vi "主VI.vi"() -> ()   [LabVIEW 2011]
panel:
  in  "长度":dbl=250.0
  out "Data":dbl[](array[numeric])
  out "Out":string=" "
  in  "退出":bool
  out "会话":u32
  in  "超时":u32=2000
  in  "地址":string="[C:DSO][D:DSO-2202M][T:USB][PID:0x834][VID:0x5656][EI:0x82][EO:0x4][CFG:1][I:0] DSO-2202M DSO-2202M"
  in  "读指令":string="dconfig;"
  in  "写指令":string="key:c1;"
  out "返回值":i32
  in  "Close":bool
  in  "Readx":bool
  in  "Writex":bool
  in  "Openx":bool
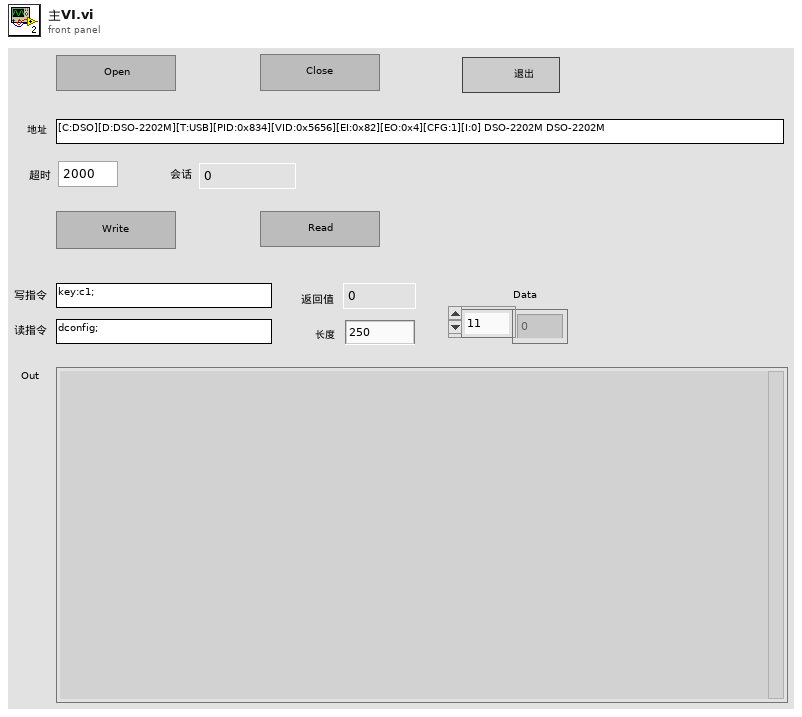
[diagram p1: front panel]
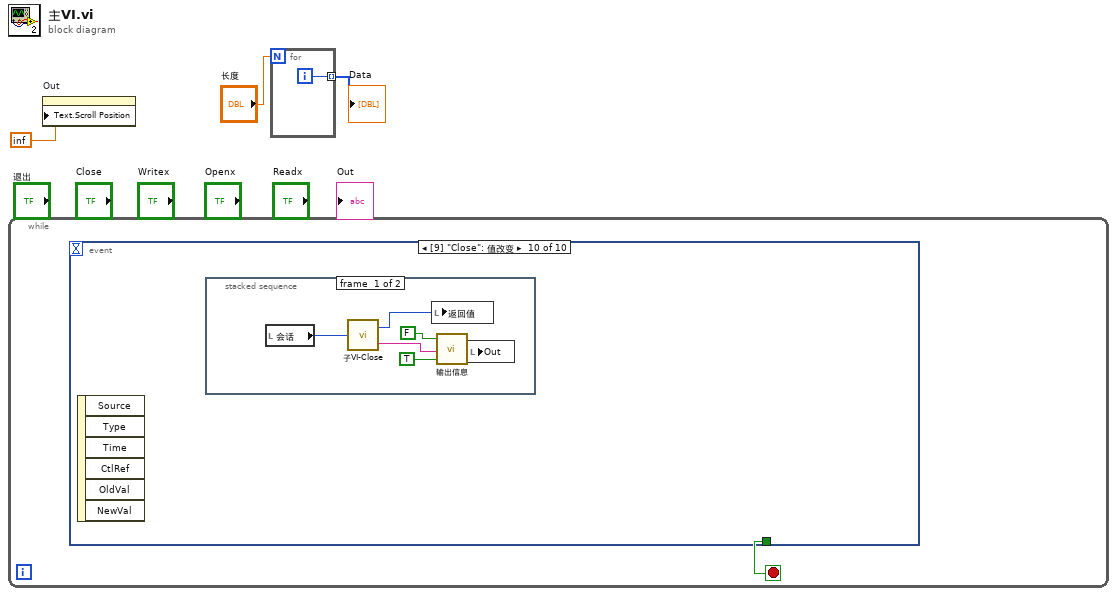
[diagram p0: block diagram]
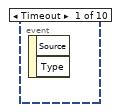
[diagram p2: hidden frame]
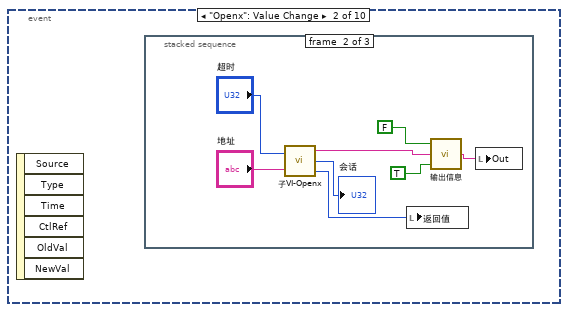
[diagram p3: hidden frame]
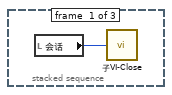
[diagram p4: hidden frame]
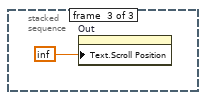
[diagram p5: hidden frame]
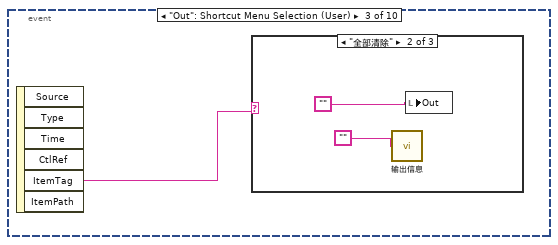
[diagram p6: hidden frame]
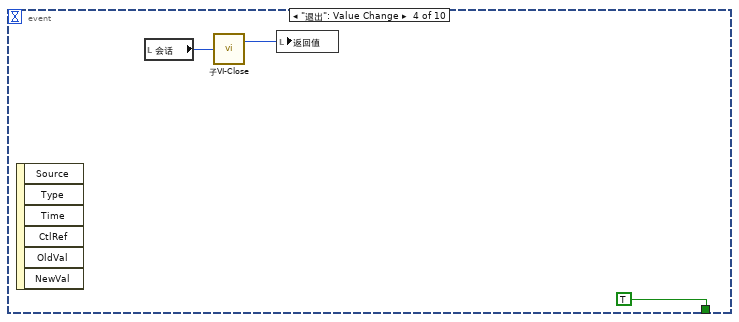
[diagram p9: hidden frame]
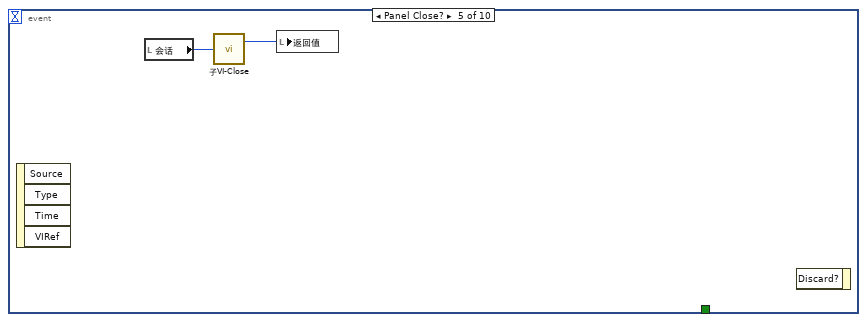
[diagram p10: hidden frame]
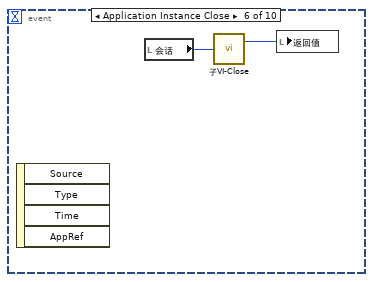
[diagram p11: hidden frame]
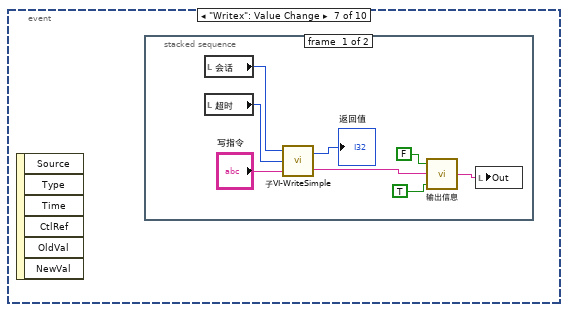
[diagram p12: hidden frame]
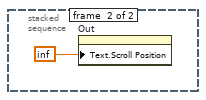
[diagram p13: hidden frame]
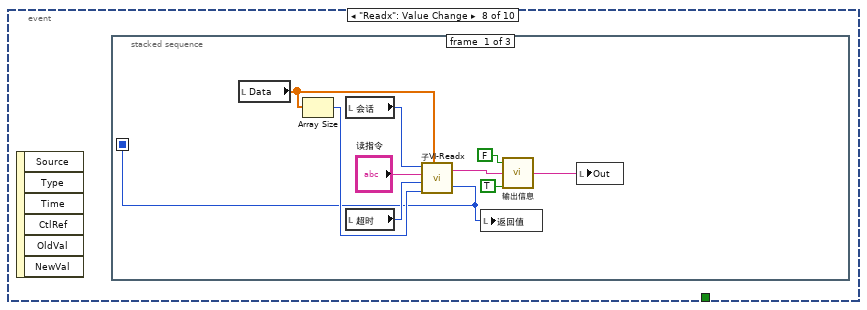
[diagram p14: hidden frame]
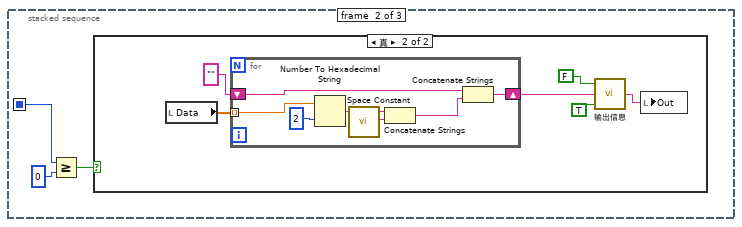
[diagram p15: hidden frame]
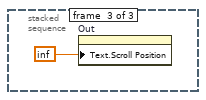
[diagram p17: hidden frame]
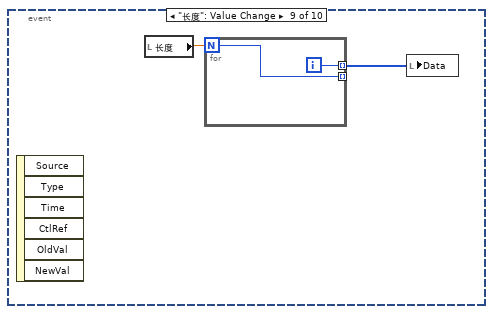
[diagram p18: hidden frame]
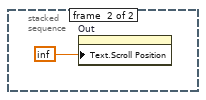
[diagram p19: hidden frame]
diagram:
  n1 = while {
    stop <- w4 stop-if-true
    n2 = event shown="[9] \"Close\": 值改变" {
      selector: _ -> [_ _ _ _ _ _ _ _ _ _]
      dyn-events: _ -> [_ _ _ _ _ _ _ _ _ _]
      timeout: _ -> [_ _ _ _ _ _ _ _ _ _]
      tunnel: [_ _ _ TRUE _ _ _ _ _ _] -> w4
      event Timeout {
        n3 = event-data() -> ()  [unwired: 1 in, 2 out]
      }
      event "Openx": Value Change {
        n4 = event-data() -> ()  [unwired: 1 in, 6 out]
        n5 = stacked-sequence {
          frame #0 {
            n6 = local read "会话"() -> (w5:u32)
            n7 = call "子VI-Close.vi"("会话"=w5) -> ()  [unwired: 2 out]
          }
          frame #1 {
            n8 = call "子VI-Openx.vi"("超时"="超时", "地址"="地址") -> ("描述"=w6:string, "会话"=→"会话":u32, "返回值"=w10:i32)
            n9 = local write "返回值"(w10) -> ()
            n10 = call "输出信息.vi"("换行"=TRUE, "In"=w6, "清空"=FALSE) -> ("Out"=w8:string)
            n11 = local write "Out"(w8) -> ()
          }
          frame #2 {
            n12 = property on="Out" class="Str"("Text.Scroll Position"=inf) -> ()  [unwired: 2 in, 2 out]
          }
        }
      }
      event "Out": Shortcut Menu Selection (User) {
        n13 = event-data() -> ("ItemTag"=w15:string)  [unwired: 1 in, 5 out]
        n14 = case shown="\"全部清除\"" w15 {
          frame "假", Default {
          }
          frame "全部清除" {
            n15 = call "输出信息.vi"("In"="") -> ()  [unwired: 2 in, 1 out]
            n16 = local write "Out"("") -> ()
          }
          frame "真" {
          }
        }
      }
      event "退出": Value Change {
        n17 = event-data() -> ()  [unwired: 1 in, 6 out]
        n18 = local read "会话"() -> (w19:u32)
        n19 = call "子VI-Close.vi"("会话"=w19) -> ("返回值"=w18:u32)  [unwired: 1 out]
        n20 = local write "返回值"(w18) -> ()
      }
      event Panel Close? {
        n21 = event-data() -> ()  [unwired: 1 in, 4 out]
        n22 = local read "会话"() -> (w22:u32)
        n23 = call "子VI-Close.vi"("会话"=w22) -> ("返回值"=w21:u32)  [unwired: 1 out]
        n24 = local write "返回值"(w21) -> ()
        n25 = event-data() -> ()  [unwired: 2 in, 1 out]
      }
      event Application Instance Close {
        n26 = event-data() -> ()  [unwired: 1 in, 4 out]
        n27 = local read "会话"() -> (w24:u32)
        n28 = call "子VI-Close.vi"("会话"=w24) -> ("返回值"=w23:u32)  [unwired: 1 out]
        n29 = local write "返回值"(w23) -> ()
      }
      event "Writex": Value Change {
        n30 = event-data() -> ()  [unwired: 1 in, 6 out]
        n31 = stacked-sequence {
          frame #0 {
            n32 = local read "会话"() -> (w32:u32)
            n33 = local read "超时"() -> (w31:u32)
            n34 = call "子VI-WriteSimple.vi"("指令"="写指令", "超时"=w31, "会话"=w32) -> ("描述"=w27:string, "返回值"=→"返回值":i32)
            n35 = call "输出信息.vi"("换行"=TRUE, "In"=w27, "清空"=FALSE) -> ("Out"=w25:string)
            n36 = local write "Out"(w25) -> ()
          }
          frame #1 {
            n37 = property on="Out" class="Str"("Text.Scroll Position"=inf) -> ()  [unwired: 2 in, 2 out]
          }
        }
      }
      event "Readx": Value Change {
        n38 = event-data() -> ()  [unwired: 1 in, 6 out]
        n39 = stacked-sequence {
          seq-local: [w38 _ _] -> [_ w46 _]
          frame #0 {
            n40 = local read "Data"() -> (w40:dbl[])
            n41 = Array Size(array=w40) -> (size(s)=w39:i32)
            n42 = local read "会话"() -> (w43:u32)
            n43 = local read "超时"() -> (w41:u32)
            n44 = call "子VI-Readx.vi"("会话"=w43, "指令"="读指令", "超时"=w41, "长度"=w39, "数据"=w40) -> ("描述"=w36:string, "返回值"=w38:i32)
            n45 = local write "返回值"(w38) -> ()
            n46 = call "输出信息.vi"("换行"=TRUE, "In"=w36, "清空"=FALSE) -> ("Out"=w34:string)
            n47 = local write "Out"(w34) -> ()
          }
          frame #1 {
            n48 = Greater Or Equal?(x=w46, y=0) -> (x >= y?=w44:bool)
            n49 = case shown="真" w44 {
              frame False {
              }
              frame True {
                n50 = local read "Data"() -> (w51:dbl[])
                n51 = for {
                  tunnel: w51 -> [w58] mode=indexing
                  shift-right: [w57] -> w49
                  shift-left: "" -> [w59]
                  n52 = Number To Hexadecimal String(1:u8 2, 2:w58) -> (0:w56:string)
                  n53 = call <vilib>:"Space Constant.vi"() -> ("String"=w55:string)
                  n54 = Concatenate Strings(w56, w55) -> (w54:string)
                  n55 = Concatenate Strings(w59, w54) -> (w57:string)
                }
                n56 = call "输出信息.vi"("换行"=TRUE, "In"=w49, "清空"=FALSE) -> ("Out"=w50:string)
                n57 = local write "Out"(w50) -> ()
              }
            }
          }
          frame #2 {
            n58 = property on="Out" class="Str"("Text.Scroll Position"=inf) -> ()  [unwired: 2 in, 2 out]
          }
        }
      }
      event "长度": Value Change {
        n59 = event-data() -> ()  [unwired: 1 in, 6 out]
        n60 = local read "长度"() -> (w61:dbl)
        n61 = for {
          N: w61 -> [w63]
          tunnel: [w64] -> w62 mode=indexing
          tunnel: [w63] -> _ mode=indexing
          i -> [w64]
        }
        n62 = local write "Data"(w62) -> ()
      }
      event "Close": Value Change {
        n63 = event-data() -> ()  [unwired: 1 in, 6 out]
        n64 = stacked-sequence {
          frame #0 {
            n65 = local read "会话"() -> (w69:u32)
            n66 = call "子VI-Close.vi"("会话"=w69) -> ("返回值"=w70:u32, "描述"=w67:string)
            n67 = local write "返回值"(w70) -> ()
            n68 = call "输出信息.vi"("换行"=TRUE, "In"=w67, "清空"=FALSE) -> ("Out"=w68:string)
            n69 = local write "Out"(w68) -> ()
          }
          frame #1 {
            n70 = property on="Out" class="Str"("Text.Scroll Position"=inf) -> ()  [unwired: 2 in, 2 out]
          }
        }
      }
    }
  }
  n71 = property on="Out" class="Str"("Text.Scroll Position"=inf) -> ()  [unwired: 2 in, 2 out]
  n72 = for {
    N: "长度" -> [_]
    tunnel: [w72] -> w2 mode=indexing
    i -> [w72]
  }
  "Data" <- w2
